vi "VIH ProjFile - HHP Generation - Read.vi"(8 "error in":errorcluster, 9 "Build Root Folder":path, 10 "Project Folder":path, 11 "XML Parent Item":refnum<k20>) -> (0 "error out":errorcluster, 1 "HHP_Generation out":T1={"HHP_Template"=enum."default", "HHP_Template_CustomPath"=path "", "HHP_Target"=enum."default", "HHP_Target_CustomPath"=path "", "HHP_CreateTOC"=TRUE, "HHP_CreateIDX"=TRUE, "HHP_DefaultTopic"=enum."auto", "HHP_DefaultTopic_CustomPath"=path "", "CHM_Filename"=path "", "HHP_AutoBuild"=FALSE, "CHM_AutoBuild"=FALSE}, 3 "dup XML Parent Item":refnum<k20>)   [LabVIEW 2014]
doc: "::: VI Helpeks :::\nCopyright (c) 2000-2026 Konstantin Shifershteyn. All rights reserved."
uses:
  _VIH CHM Project.llb/VIH - CHM Project - HHP Generation Params Cluster.ctl
  <vilib>/xml/Close Reference(Node).vi
  <vilib>/xml/NI_XML.lvlib
panel:
  in  "HHP_Generation (data)":T1={"HHP_Template"=enum."default", "HHP_Template_CustomPath"=path "", "HHP_Target"=enum."default", "HHP_Target_CustomPath"=path "", "HHP_CreateTOC"=TRUE, "HHP_CreateIDX"=TRUE, "HHP_DefaultTopic"=enum."auto", "HHP_DefaultTopic_CustomPath"=path "", "CHM_Filename"=path "", "HHP_AutoBuild"=FALSE, "CHM_AutoBuild"=FALSE}
  # "VI Helpeks\nCopyright (c) 2012-2026 Konstantin Shifershteyn"
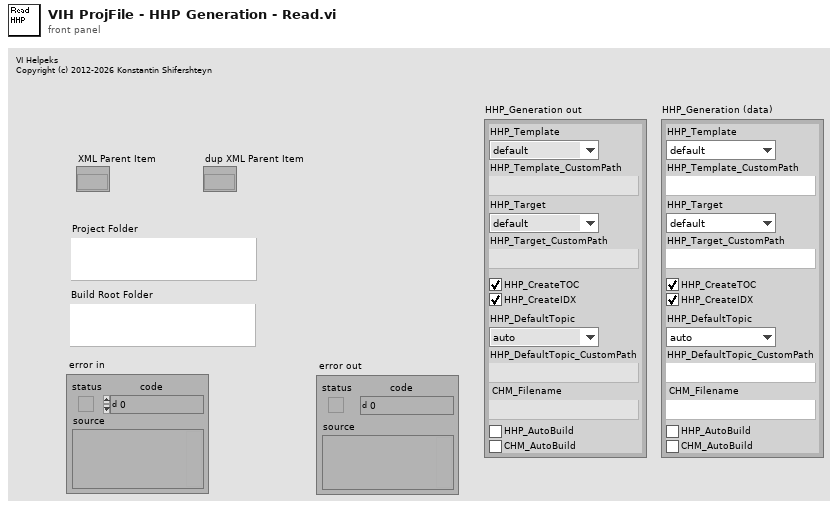
[diagram p1: front panel]
types:
  T1 = typedef "VIH - CHM Project - HHP Generation Params Cluster.ctl" = cluster{"HHP_Template":enum16{"default", "custom"}, "HHP_Template_CustomPath":path, "HHP_Target":enum16{"default", "custom"}, "HHP_Target_CustomPath":path, "HHP_CreateTOC":bool, "HHP_CreateIDX":bool, "HHP_DefaultTopic":enum16{"auto", "custom"}, "HHP_DefaultTopic_CustomPath":path, "CHM_Filename":path, "HHP_AutoBuild":bool, "CHM_AutoBuild":bool}
  T2 = typedef "CHM Project - HHP Generation Params Cluster.ctl" = cluster{"HHP_Template":enum16{"default", "custom"}, "HHP_Template_CustomPath":path, "HHP_Target":enum16{"default", "custom"}, "HHP_Target_CustomPath":path, "HHP_CreateTOC":bool, "HHP_CreateIDX":bool, "HHP_DefaultTopic":enum16{"auto", "custom"}, "HHP_DefaultTopic_CustomPath":path, "CHM_Filename":path, "HHP_AutoBuild":bool, "CHM_AutoBuild":bool}
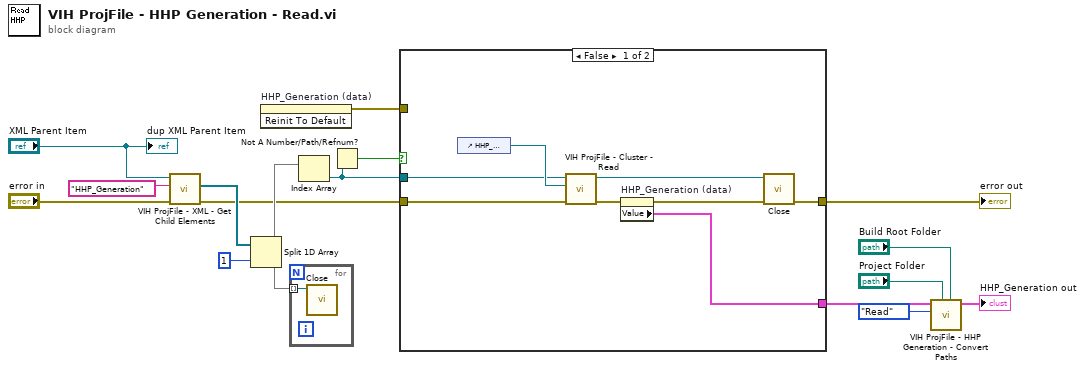
[diagram p0: block diagram]
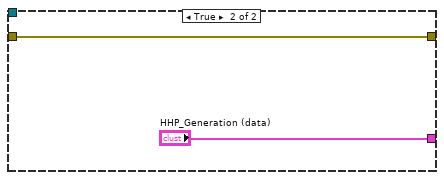
[diagram p2: hidden frame]
diagram:
  n1 = call "VIH ProjFile - XML - Get Child Elements.vi"("error in"="error in", "Tag Name"="HHP_Generation", "XML Parent Item"="XML Parent Item") -> ("error out"=w3:errorcluster, "Array of Elements"=w10:refnum<k20>[])  [unwired: 6 in, 1 out]
  n2 = Split 1D Array(array=w10, index=1) -> (first subarray=w13:refnum<k20>[], second subarray=w12:refnum<k20>[])
  n3 = invoke on="HHP_Generation (data)" class="Clust (strict)" method="Reinit To Default"() -> (error out=w2:errorcluster)  [unwired: 3 in, 2 out]
  n4 = for {
    tunnel: w12 -> [w18] mode=indexing
    n5 = call-poly <vilib>:"Close.vi"("node"=w18) -> ()  [unwired: 8 in, 1 out]
  }
  n6 = Index Array(array=w13) -> (element=w16:refnum<k20>)  [unwired: 1 in]
  n7 = Not A Number/Path/Refnum?(number/path/refnum=w16) -> (NaN/Path/Refnum?=w15:bool)
  n8 = case shown="False" w15 {
    tunnel: w3 -> [w19 w28]
    tunnel: [w25 w28] -> w17
    tunnel: [w20 "HHP_Generation (data)"] -> w5
    tunnel: w16 -> [w23 _]
    tunnel: w2 -> [_ _]
    frame False {
      n9 = control-ref of="HHP_Generation (data)"() -> (w26:refnum<vi>)
      n10 = call "VIH ProjFile - Cluster - Read.vi"("error in"=w19, "Ctl Refnum"=w26, "XML Parent Item"=w23) -> ("error out"=w24:errorcluster, "dup XML Parent Item"=w22:refnum<k20>)  [unwired: 7 in]
      n11 = property on="HHP_Generation (data)" class="Clust (strict)"(error in=w24) -> (error out=w21:errorcluster, "Value"=w20:T2)  [unwired: 1 in, 1 out]
      n12 = call-poly <vilib>:"Close.vi"("error in (no error)"=w21, "node"=w22) -> ("error out"=w25:errorcluster)  [unwired: 7 in]
    }
    frame True {
    }
  }
  "error out" <- w17
  n13 = call "VIH ProjFile - HHP Generation - Convert Paths.vi"("Build Root Dir"="Build Root Folder", "Project Dir"="Project Folder", "Operation"=enum16{"Read", "Write"}."Read", "HHP_Generation"=w5) -> ("HHP_Generation out"=→"HHP_Generation out":T1)  [unwired: 7 in]
  "dup XML Parent Item" <- "XML Parent Item"
